vi "Accumulator.vi"(0 "N":i32=5) -> (1 "Sum":i32, 2 "SumSq":i32, 3 "Product":i32, 4 "Done":bool)   [LabVIEW 2026]
doc: "Round17 complex-demo flagship: a While Loop with four shift registers accumulating, over N iterations (element = iteration index + 1), the running Sum, Sum of Squares, and Product. Demonstrates AI-authored loops, shift registers, arithmetic, and conditional termination - a genuinely algorithmic VI - built and run through the pylabview backend (no gRPC/Nigel required). Verified for N=5: Sum=15, SumSq=55, Product=120, Done=true. Constants feeding shift-register terminals stay on the root diagram; constants feeding loop-internal arithmetic enter via Tunnels (LV012)."
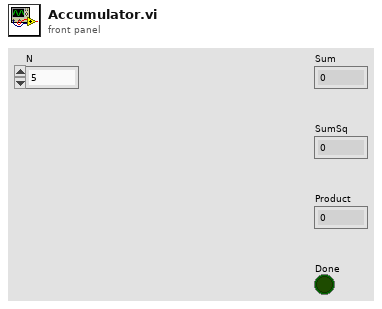
[diagram p1: front panel]
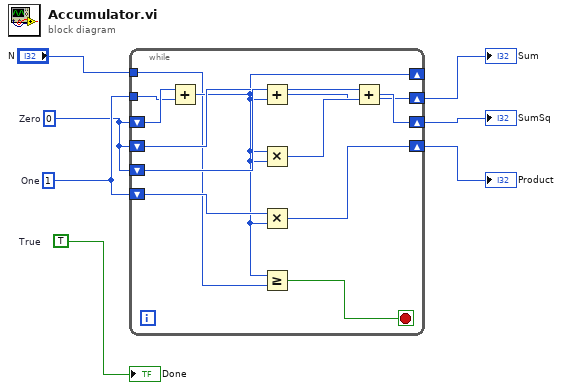
[diagram p0: block diagram]
diagram:
  w4 = TRUE  # True
  w3 = 1  # One
  w2 = 0  # Zero
  n1 = while {
    tunnel: "N" -> [w8]
    tunnel: w3 -> [w9]
    shift-right: [w11] -> _
    shift-left: w2 -> [w10]
    shift-right: [w13] -> w5
    shift-left: w2 -> [w12]
    shift-right: [w15] -> w6
    shift-left: w2 -> [w14]
    shift-right: [w17] -> w7
    shift-left: w3 -> [w16]
    stop <- w19 stop-if-true
    n2 = Add(x=w10, y=w9) -> (x+y=w11:i32)
    n3 = Add(x=w12, y=w11) -> (x+y=w13:i32)
    n4 = Multiply(x=w11, y=w11) -> (x*y=w18:i32)
    n5 = Multiply(x=w16, y=w11) -> (x*y=w17:i32)
    n6 = Greater Or Equal?(x=w11, y=w8) -> (x >= y?=w19:bool)
    n7 = Add(x=w14, y=w18) -> (x+y=w15:i32)
  }
  "Sum" <- w5
  "SumSq" <- w6
  "Product" <- w7
  "Done" <- w4
